vi "Set Cell Column Span.vi"(7 "Range":i32, 8 "error in":errorcluster, 9 "Column":i32, 10 "Row":i32, 11 "SourceGrid in":refnum<class "SourceGrid.lvclass">) -> (0 "error out":errorcluster, 3 "SourceGrid out":refnum<class "SourceGrid.lvclass">)   [LabVIEW 2020, in "SourceGrid.lvlib" / "SourceGrid.lvclass"]
doc: "ColSpan for merge operation, calculated using the current range."
uses:
  SourceGrid.lvclass
  SourceGrid.lvclass/SourceGrid.ctl
  D:/git/Sourcegrid-LabVIEW/source/SourceGrid.dll
  SourceGrid.dll
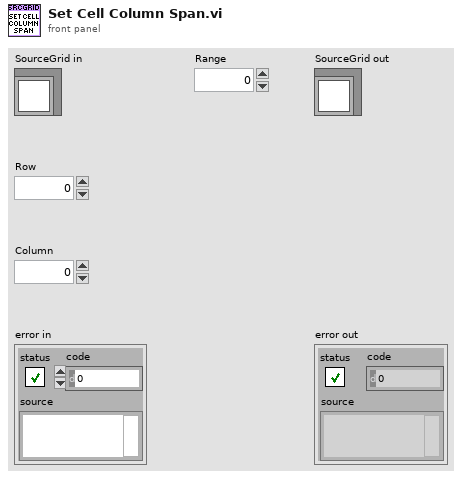
[diagram p1: front panel]
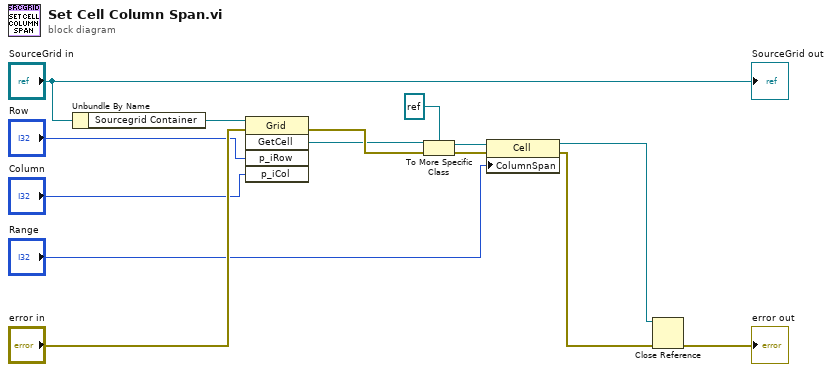
[diagram p0: block diagram]
diagram:
  n1 = Unbundle By Name("SourceGrid in") -> ("Sourcegrid Container"=w13:refnum<k24>)
  n2 = invoke class="Grid" method="GetCell"(reference=w13, error in="error in", "p_iRow"="Row", "p_iCol"="Column") -> (error out=w11:errorcluster, "GetCell"=w4:refnum<k24>)  [unwired: 1 in, 3 out]
  n3 = To More Specific Class(target class=refnum<k24> refnum ("new reference"), reference=w4, error in=w11) -> (specific class reference=w3:refnum<k24>, error out=w8:errorcluster)
  n4 = property class="Cell"(reference=w3, error in=w8, "ColumnSpan"="Range") -> (reference out=w1:refnum<k24>, error out=w5:errorcluster)
  n5 = Close Reference(reference=w1, error in (no error)=w5) -> (error out=→"error out":errorcluster)
  "SourceGrid out" <- "SourceGrid in"
